vi "RDC-test-get_perm.vi"() -> ()   [LabVIEW 2020]
doc: "Test panel, run by hand: computes the permittivity with the DAK 3.5 probe values and the linear correction VIs and shows the error against reference data."
uses:
  RDC-error_metric_clust.ctl
  Reflector/RFH-common_data_format.ctl
  RDC-Reflection_Data_Computation.lvlib
  Reflector/RFH-Reflection_File_Handler.lvlib
panel:
  in  "Enable bruteforce offset":bool
  out "element":string
  in  "Tab Control":enum32{"Compare", "Impedance", "Error Check"}(tab)
  out "Real Perm":T1(graph)
  out "Tau":dbl format="%#_6p"
  out "C0":dbl format="%#_6p"
  out "Imag Perm":T1(graph)
  out "Reactance":cluster{"Frequency":dbl[], dbl[]}(graph)
  out "Resistance":cluster{"Frequency":dbl[], dbl[]}(graph)
  out "Diff Real":dbl[](graph)
  out "Diff Imag":dbl[](graph)
  out "percent diff real":dbl[](graph)
  out "percent diff imag":dbl[](graph)
  out "Error Metric":T2
  in  "Numeric":i32=3
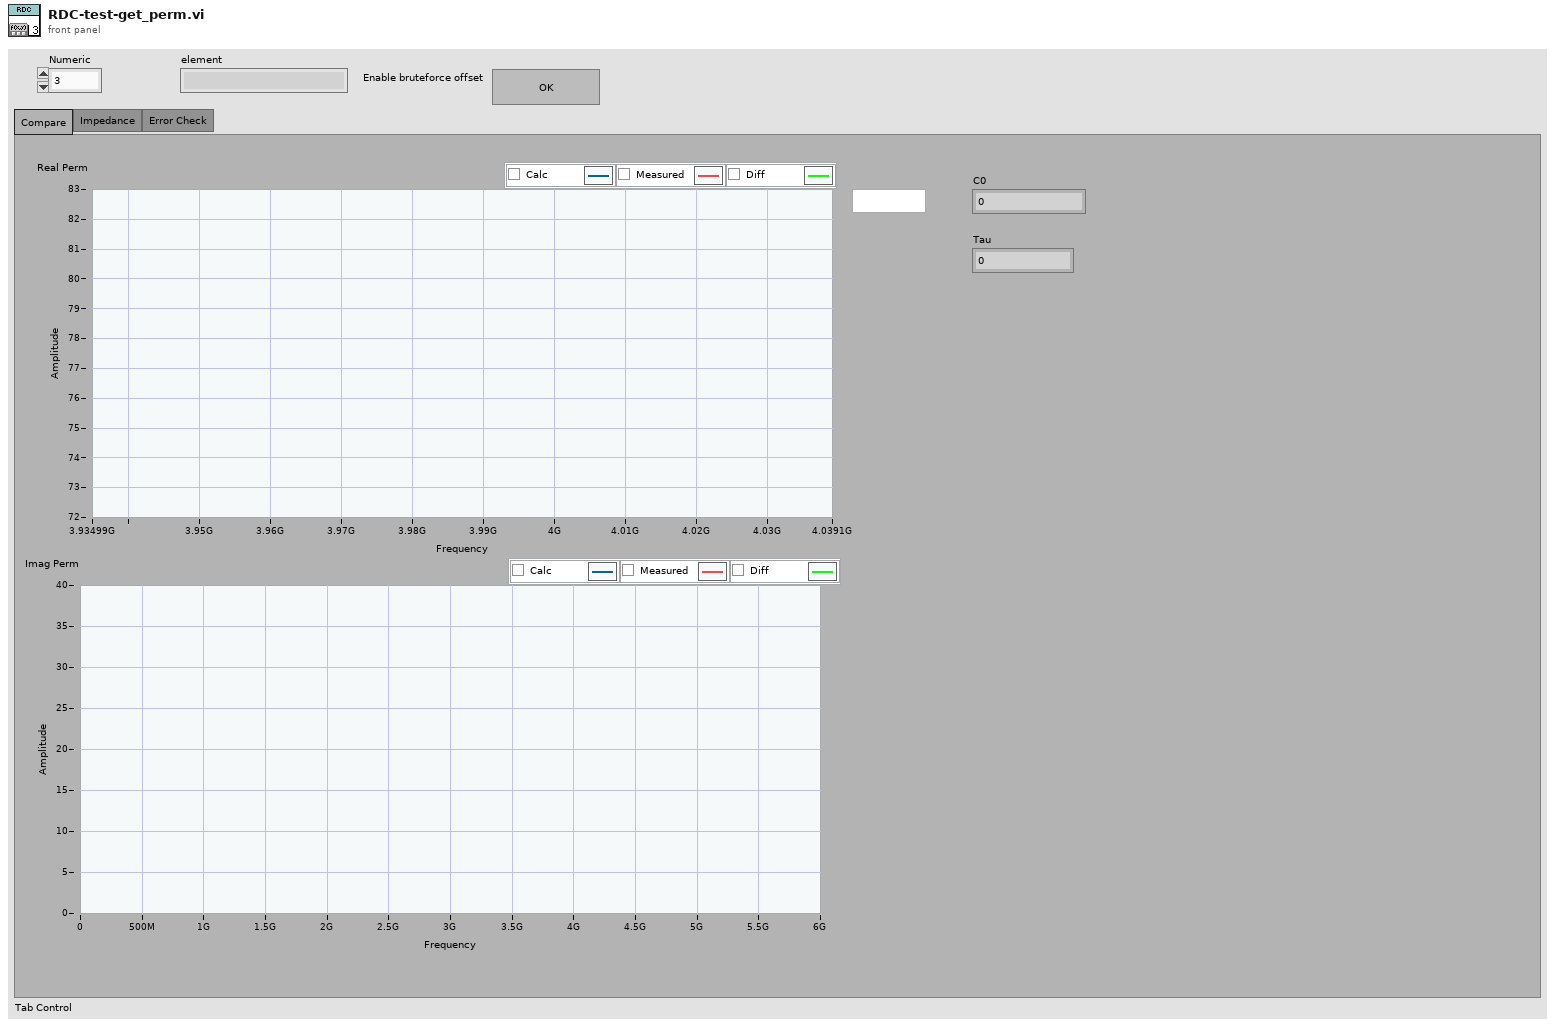
[diagram p1: front panel]
types:
  T1 = cluster{"Frequency":dbl[], "Permativity'":dbl[]}[]
  T2 = typedef "RDC-Reflection_Data_Computation.lvlib/RDC-error_metric_clust.ctl" = cluster{"Diff":cdb[], "percent diff":cdb[], "Average diff":cdb, "Percent avg diff":cdb, "RMSE diff":cdb}
  T3 = typedef "RFH-Reflection_File_Handler.lvlib/RFH-common_data_format.ctl" = cluster{"Frequency":dbl[], "Reflection'":dbl[], "Reflection''":dbl[], "Permativity'":dbl[], "Permativity''":dbl[], "Conductivity":dbl[], "Loss Tangent":dbl[], "Resistance":dbl[], "Reactance":dbl[]}
  T4 = cluster{"Frequency":dbl[], "Permativity''":dbl[]}
  T5 = cluster{"Frequency":dbl[], "Permativity''":dbl[]}[]
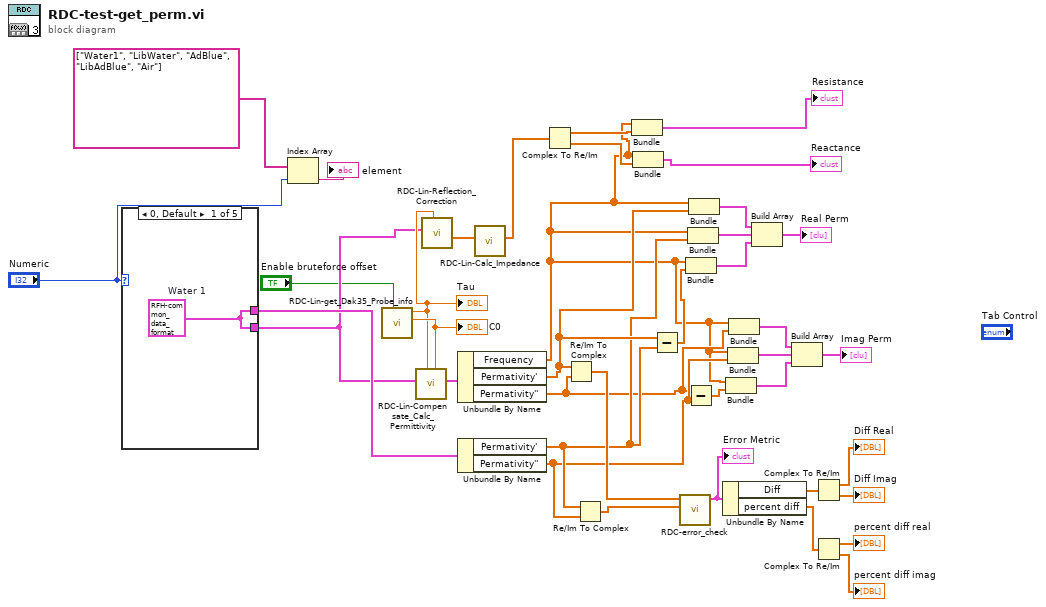
[diagram p0: block diagram]
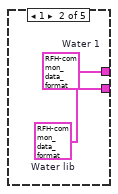
[diagram p2: hidden frame]
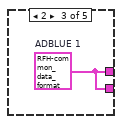
[diagram p3: hidden frame]
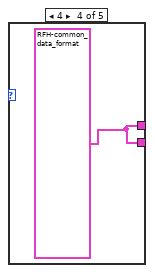
[diagram p4: hidden frame]
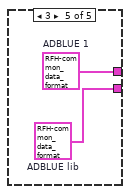
[diagram p5: hidden frame]
diagram:
  n1 = case shown="0, Default" "Numeric" {
    tunnel: [w40 w41 w43 w44 w46] -> w8
    tunnel: [w40 w42 w43 w44 w45] -> w37
    frame 0, Default {
      w40 = T3 {"Frequency"=array[2001 elements], "Reflection'"=array[2001 elements], "Reflection''"=array[2001 elements], "Permativity'"=array[2001 elements], "Permativity''"=array[2001 elements], "Conductivity"=array[2001 elements], "Loss Tangent"=array[2001 elements], "Resistance"=[], "Reactance"=[]}  # Water 1
    }
    frame 1 {
      w41 = T3 {"Frequency"=array[2001 elements], "Reflection'"=array[2001 elements], "Reflection''"=array[2001 elements], "Permativity'"=array[2001 elements], "Permativity''"=array[2001 elements], "Conductivity"=array[2001 elements], "Loss Tangent"=array[2001 elements], "Resistance"=[], "Reactance"=[]}  # Water lib
      w42 = T3 {"Frequency"=array[2001 elements], "Reflection'"=array[2001 elements], "Reflection''"=array[2001 elements], "Permativity'"=array[2001 elements], "Permativity''"=array[2001 elements], "Conductivity"=array[2001 elements], "Loss Tangent"=array[2001 elements], "Resistance"=[], "Reactance"=[]}  # Water 1
    }
    frame 2 {
      w43 = T3 {"Frequency"=array[2001 elements], "Reflection'"=array[2001 elements], "Reflection''"=array[2001 elements], "Permativity'"=array[2001 elements], "Permativity''"=array[2001 elements], "Conductivity"=array[2001 elements], "Loss Tangent"=array[2001 elements], "Resistance"=[], "Reactance"=[]}  # ADBLUE 1
    }
    frame 4 {
      w44 = T3 {"Frequency"=array[2001 elements], "Reflection'"=array[2001 elements], "Reflection''"=array[2001 elements], "Permativity'"=array[2001 elements], "Permativity''"=array[2001 elements], "Conductivity"=array[2001 elements], "Loss Tangent"=array[2001 elements], "Resistance"=[], "Reactance"=[]} ("Air")
    }
    frame 3 {
      w45 = T3 {"Frequency"=array[2001 elements], "Reflection'"=array[2001 elements], "Reflection''"=array[2001 elements], "Permativity'"=array[2001 elements], "Permativity''"=array[2001 elements], "Conductivity"=array[2001 elements], "Loss Tangent"=array[2001 elements], "Resistance"=[], "Reactance"=[]}  # ADBLUE 1
      w46 = T3 {"Frequency"=array[2001 elements], "Reflection'"=array[2001 elements], "Reflection''"=array[2001 elements], "Permativity'"=array[2001 elements], "Permativity''"=array[2001 elements], "Conductivity"=array[2001 elements], "Loss Tangent"=array[2001 elements], "Resistance"=[], "Reactance"=[]}  # ADBLUE lib
    }
  }
  n2 = Index Array(array=string[] ["Water1", "LibWater", "AdBlue", "LibAdBlue", "Air"], index="Numeric") -> (element=→"element":string)
  n3 = call "RDC-Lin-get_Dak35_Probe_info.vi"("Enable bruteforce offset"="Enable bruteforce offset") -> ("C0"=w39:dbl, "Tau"=w9:dbl)  [unwired: 9 in]
  "Tau" <- w9
  "C0" <- w39
  n4 = call "RDC-Lin-Compensate_Calc_Permittivity.vi"("C0"=w39, "Tau"=w9, "input cluster"=w8) -> ("Output cluster"=w38:T3)  [unwired: 8 in]
  n5 = call "RDC-Lin-Reflection_Correction.vi"("Tau"=w9, "Measured"=w8) -> ("Reflection Tip"=w10:cdb[])  [unwired: 8 in, 1 out]
  n6 = Unbundle By Name(w38) -> ("Frequency"=w4:dbl[], "Permativity'"=w24:dbl[], "Permativity''"=w11:dbl[])
  n7 = Unbundle By Name(w37) -> ("Permativity'"=w23:dbl[], "Permativity''"=w12:dbl[])
  n8 = call "RDC-Lin-Calc_Impedance.vi"("Reflection Tip"=w10) -> ("Impedance"=w7:cdb[])  [unwired: 9 in, 1 out]
  n9 = Complex To Re/Im(x + iy=w7) -> (x=w6:dbl[], y=w5:dbl[])
  n10 = Re/Im To Complex(1:w11, 2:w24) -> (0:w30:cdb[])
  n11 = Re/Im To Complex(1:w12, 2:w23) -> (0:w28:cdb[])
  n12 = Bundle("Frequency"=w4, w6) -> (→"Resistance":cluster{"Frequency":dbl[], dbl[]})  [unwired: 1 in]
  n13 = Bundle("Frequency"=w4, w5) -> (→"Reactance":cluster{"Frequency":dbl[], dbl[]})  [unwired: 1 in]
  n14 = Subtract(x=w24, y=w23) -> (x-y=w18:dbl[])
  n15 = call "RDC-error_check.vi"("Reference"=w28, "Calculated"=w30) -> ("Error Metric"=w29:T2)  [unwired: 9 in]
  "Error Metric" <- w29
  n16 = Bundle("Frequency"=w4, w18) -> (w20:cluster{"Frequency":dbl[], dbl[]})  [unwired: 1 in]
  n17 = Subtract(x=w11, y=w12) -> (x-y=w13:dbl[])
  n18 = Bundle("Frequency"=w4, "Permativity'"=w23) -> (w21:cluster{"Frequency":dbl[], "Permativity'":dbl[]})  [unwired: 1 in]
  n19 = Bundle("Frequency"=w4, "Permativity'"=w24) -> (w22:cluster{"Frequency":dbl[], "Permativity'":dbl[]})  [unwired: 1 in]
  n20 = Unbundle By Name(w29) -> ("Diff"=w31:cdb[], "percent diff"=w32:cdb[])
  n21 = Bundle("Frequency"=w4, w13) -> (w16:cluster{"Frequency":dbl[], dbl[]})  [unwired: 1 in]
  n22 = Bundle("Frequency"=w4, "Permativity''"=w12) -> (w15:T4)  [unwired: 1 in]
  n23 = Bundle("Frequency"=w4, "Permativity''"=w11) -> (w14:T4)  [unwired: 1 in]
  n24 = Build Array(w22, w21, w20) -> (→"Real Perm":T1)
  n25 = Build Array(w14, w15, w16) -> (→"Imag Perm":T5)
  n26 = Complex To Re/Im(x + iy=w31) -> (x=→"Diff Real":dbl[], y=→"Diff Imag":dbl[])
  n27 = Complex To Re/Im(x + iy=w32) -> (x=→"percent diff real":dbl[], y=→"percent diff imag":dbl[])
